vi "VIH Project - Change Flag.vi"(11 "cmd (get)":enum16{"get", "set", "reset"}(ring)) -> (2 "Counter":i32, 3 "Flag":bool)   [LabVIEW 2014]
doc: "::: VI Helpeks :::\nCopyright (c) 2000-2026 Konstantin Shifershteyn. All rights reserved."
panel:
  # "VI Helpeks\nCopyright (c) 2012-2026 Konstantin Shifershteyn"
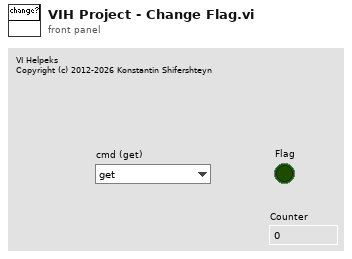
[diagram p1: front panel]
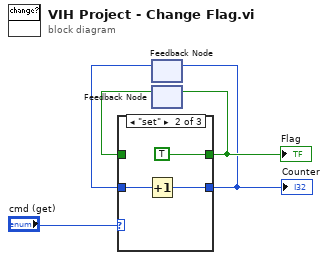
[diagram p0: block diagram]
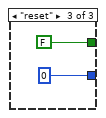
[diagram p3: hidden frame]
diagram:
  n1 = feedback #1() -> (w2:i32)  [unwired: 1 in]
  n2 = feedback #2() -> (w4:bool)  [unwired: 1 in]
  n3 = case shown="\"set\"" "cmd (get)" {
    tunnel: [w7 TRUE FALSE] -> w3
    tunnel: w4 -> [w7 _ _]
    tunnel: [w6 w8 0] -> w1
    tunnel: w2 -> [w6 w9 _]
    frame "get" {
    }
    frame "set" {
      n4 = Increment(x=w9) -> (x+1=w8:i32)
    }
    frame "reset" {
    }
  }
  "Flag" <- w3
  "Counter" <- w1
  n5 = feedback-in #1(w1) -> ()
  n6 = feedback-in #2(w3) -> ()
